vi "Forward Packet.vi"(10 "Response":T1, 11 "Session in":refnum<class "Session.lvclass">) -> (0 "error out":errorcluster)   [LabVIEW 2013, in "MQTT Base.lvlib" / "Session.lvclass"]
uses:
  Session.lvclass
  Base Class/Response -- cluster.ctl
  <vilib>/LabVIEW Open Source Project/MQTT Control Packets/Control Packets/ControlPacket/ControlPacket.lvclass
  Pending ACKs -- cluster.ctl
  Session.lvclass/Session.ctl
  Session Disconnection Reason -- enum.ctl
  DebuggingTerminal/Stream Direction -- enum.ctl
  <vilib>/LabVIEW Open Source Project/Connection/Connection/Connection.lvclass
  DebuggingTerminal/DebuggingTerminal.lvclass
  Base Class/MQTT_Base.lvclass
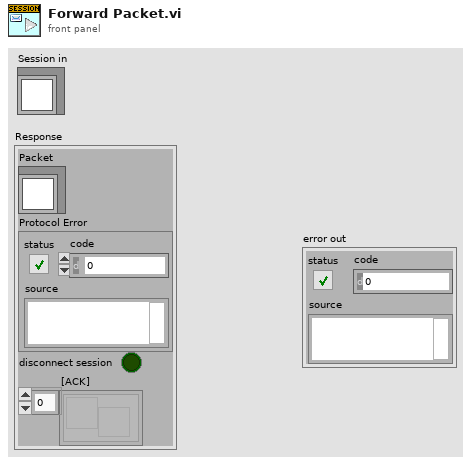
[diagram p1: front panel]
types:
  T1 = typedef "MQTT Base.lvlib/MQTT_Base.lvclass/Response -- cluster.ctl" = cluster{"Packet":refnum<class "ControlPacket.lvclass">, "Protocol Error":errorcluster, "disconnect session":bool, "[ACK]":refnum<notifier>[]}
  T2 = typedef "MQTT Base.lvlib/Session.lvclass/Pending ACKs -- cluster.ctl" = cluster{"Message":refnum<class "ControlPacket.lvclass">, "[ACK]":refnum<notifier>[], "Packet Identifier":u32}
  T3 = typedef "MQTT Base.lvlib/Session.lvclass/Session Disconnection Reason -- enum.ctl" = enum16{"Normal Stop", "Protocol Violation", "Disconnected by Peer"}
  T4 = typedef "MQTT Base.lvlib/DebuggingTerminal.lvclass/Stream Direction -- enum.ctl" = enum16{"Incoming", "Outgoing"}
  T5 = typedef "MQTT_Control_Packets.lvlib/ControlPacket.lvclass/Control Packet Type -- enum.ctl" = enum16{"Reserved", "CONNECT", "CONNACK", "PUBLISH", "PUBACK", "PUBREC", "PUBREL", "PUBCOMP", "SUBSCRIBE", "SUBACK", "UNSUBSCRIBE", "UNSUBACK", "PINGREQ", "PINGRESP", "DISCONNECT", "AUTH"}
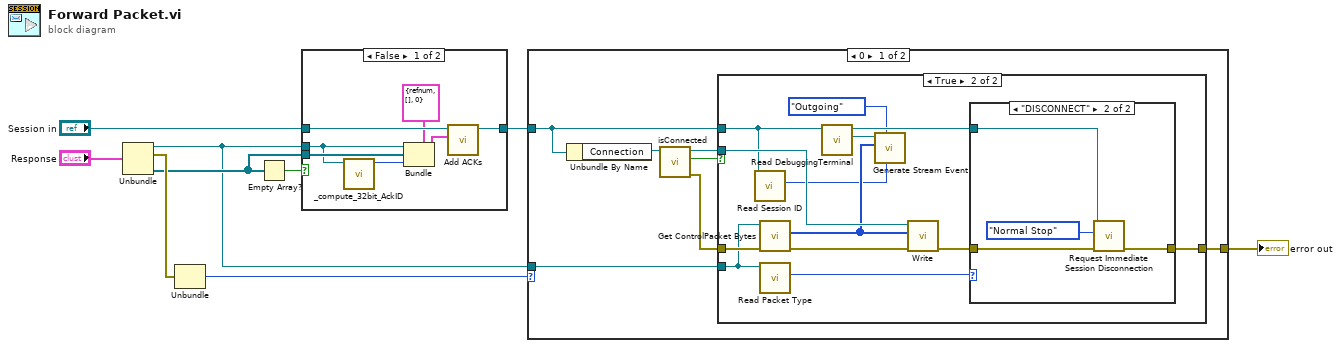
[diagram p0: block diagram]
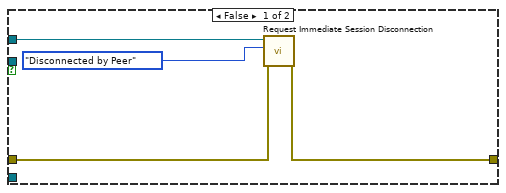
[diagram p2: hidden frame]
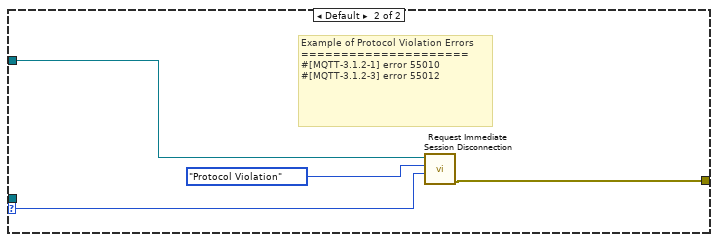
[diagram p4: hidden frame]
diagram:
  n1 = Unbundle("Response") -> ("Packet"=w1:refnum<class "ControlPacket.lvclass">, "Protocol Error"=w8:errorcluster, "[ACK]"=w7:refnum<notifier>[])  [unwired: 1 out]
  n2 = Unbundle(w8) -> ("code"=w3:i32)  [unwired: 2 out]
  n3 = Empty Array?(array=w7) -> (empty?=w2:bool)
  n4 = case shown="False" w2 {
    tunnel: "Session in" -> [w16 w17]
    tunnel: [w15 w17] -> w9
    tunnel: w1 -> [w11 _]
    tunnel: w7 -> [w14 _]
    frame False {
      n5 = call "_compute_32bit_AckID.vi"("ControlPacket in"=w11) -> ("ACK ID"=w10:u32)  [unwired: 10 in]
      n6 = Bundle(cluster=T2 {"Message"=refnum, "[ACK]"=[], "Packet Identifier"=0} ("Pending ACK"), "Message"=w11, "[ACK]"=w14, "Packet Identifier"=w10) -> (w13:T2)
      n7 = call "Add ACKs.vi"("Pending ACK"=w13, "Session in"=w16) -> ("Session out"=w15:refnum<class "Session.lvclass">)  [unwired: 8 in, 1 out]
    }
    frame True {
      # "No Acks."
    }
  }
  n8 = case shown="0" w3 {
    selector: w3 -> [_ w47]
    tunnel: w9 -> [w22 w49]
    tunnel: [w24 w48] -> w4
    tunnel: w1 -> [w23 _]
    frame 0 {
      n9 = Unbundle By Name(w22) -> ("Connection"=w21:refnum<class "Connection.lvclass">)
      n10 = call <vilib>:"isConnected.vi"("Connection in"=w21) -> ("error out"=w19:errorcluster, "connected"=w20:bool, "Connection out"=w18:refnum<class "Connection.lvclass">)  [unwired: 8 in]
      n11 = case shown="True" w20 {
        tunnel: [w25 w40] -> w24
        tunnel: w23 -> [_ w39]
        tunnel: w18 -> [_ w37]
        tunnel: w19 -> [w26 w41]
        tunnel: w22 -> [w27 w30]
        frame False {
          n12 = call "Request Immediate Session Disconnection.vi"("error in (no error)"=w26, "Disconnection Reason"=Session_Disconnection_Reason_--_enum."Disconnected by Peer", "Session in"=w27) -> ("error out"=w25:errorcluster)  [unwired: 7 in, 1 out]
        }
        frame True {
          n13 = call "Read Session ID.vi"("Session in"=w30) -> ("Session ID"=w29:i32)  [unwired: 8 in, 2 out]
          n14 = call <vilib>:"Get ControlPacket Bytes.vi"("error in (no error)"=w41, "ControlPacket"=w39) -> ("error out"=w36:errorcluster, "Bytes Stream"=w32:u8[])  [unwired: 6 in, 2 out]
          n15 = call <vilib>:"Read Packet Type.vi"("ControlPacket in"=w39) -> ("Control Packet Type"=w38:T5)  [unwired: 9 in, 1 out]
          n16 = call "Read DebuggingTerminal.vi"("Session in"=w30) -> ("DebuggingTerminal"=w33:refnum<class "DebuggingTerminal.lvclass">, "Session out"=w34:refnum<class "Session.lvclass">)  [unwired: 8 in, 1 out]
          n17 = call "Generate Stream Event.vi"("Session ID"=w29, "Direction"=Stream_Direction_--_enum."Outgoing", "Bytes"=w32, "DebuggingTerminal in"=w33) -> ()  [unwired: 6 in, 2 out]
          n18 = call <vilib>:"Write.vi"("error in (no error)"=w36, "Bytes"=w32, "Connection in"=w37) -> ("error out"=w35:errorcluster)  [unwired: 7 in, 1 out]
          n19 = case shown="\"DISCONNECT\"" w38 {
            tunnel: w34 -> [_ w45]
            tunnel: w35 -> [w42 w44]
            tunnel: [w42 w43] -> w40
            frame Default {
            }
            frame "DISCONNECT" {
              n20 = call "Request Immediate Session Disconnection.vi"("error in (no error)"=w44, "Disconnection Reason"=Session_Disconnection_Reason_--_enum."Normal Stop", "Session in"=w45) -> ("error out"=w43:errorcluster)  [unwired: 7 in, 1 out]
            }
          }
        }
      }
    }
    frame Default {
      # "Example of Protocol Violation Errors\n=====================\n#[MQTT-3.1.2-1] error 55010\n#[MQTT-3.1.2-3] error 55012"
      n21 = call "Request Immediate Session Disconnection.vi"("Protocol Violation Error Code"=w47, "Disconnection Reason"=Session_Disconnection_Reason_--_enum."Protocol Violation", "Session in"=w49) -> ("error out"=w48:errorcluster)  [unwired: 7 in, 1 out]
    }
  }
  "error out" <- w4
